vi "Teleop.vi"(10 "Match Info":T1={"Autonomous Elapsed Seconds"=0.0, "TeleOp Elapsed Seconds"=0.0, "Disabled Elapsed Seconds"=0.0, "Visited Autonomous"=FALSE, "Visited TeleOp"=FALSE, "Visited Disabled"=FALSE, "Autonomous Settings"={"Autonomous Style"=enum."Independent", "VI Refnum"=refnum}}, 11 "Call Context":T2) -> ()   [LabVIEW 2018]
doc: "This VI is called for each TeleOp packet received from the DS where the robot is not disabled. It is often used to read from the joysticks and update I/O or to update setpoints for timed control loops. It should complete and return within 20 milliseconds or it may miss DS packets."
uses:
  <vilib>/Rock Robotics/WPI/DriverStation/WPI_DriverStationDerivedRobotMode.ctl
  <vilib>/Rock Robotics/WPI/DriverStation/WPI_DriverStationMatch Info.ctl
  <vilib>/Rock Robotics/WPI/ThirdParty/Phoenix-LabVIEW/Motor Controller/Controls/CTRE_Phoenix_MotorControl_ControlMode.ctl
  <vilib>/Rock Robotics/WPI/Utilities/WPI_GetSetVariantRefNum.vi
  <vilib>/Rock Robotics/Network Tables/NT Write Boolean Array.vi
  <vilib>/Rock Robotics/Network Tables/NT Write Numeric Array.vi
  <vilib>/Rock Robotics/Network Tables/NT Write Number.vi
  Global 1.vi
panel:
  out "motor value after \nalex program":dbl
  out "slider value input":dbl
  # "r"
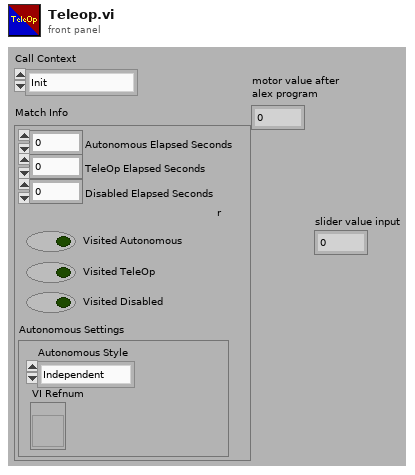
[diagram p1: front panel]
types:
  T1 = typedef "WPI_DriverStationMatch Info.ctl" = cluster{"Autonomous Elapsed Seconds":dbl, "TeleOp Elapsed Seconds":dbl, "Disabled Elapsed Seconds":dbl, "Visited Autonomous":bool, "Visited TeleOp":bool, "Visited Disabled":bool, "Autonomous Settings":cluster{"Autonomous Style":enum16{"Iterative", "Independent"}, "VI Refnum":refnum<vi>}}
  T2 = typedef "WPI_DriverStationDerivedRobotMode.ctl" = enum16{"Init", "Execute", "Stop"}
  T3 = typedef "WPI_JoystickDevRef.ctl" = cluster{"Device":T4}
  T4 = typedef "WPI_JoystickDeviceEnum.ctl" = enum16{"USB 0", "USB 1", "USB 2", "USB 3", "USB 4", "USB 5"}
  T5 = typedef "WPI_SwitchDevRef.ctl" = cluster{"DevStatus":errorcluster, "DIO Channel":T6, "CntIndex":T7, "Normally Closed":bool}
  T6 = typedef "FPGA_DIOChannel.ctl" = enum8{"DIO 0", "DIO 1", "DIO 2", "DIO 3", "DIO 4", "DIO 5", "DIO 6", "DIO 7", "DIO 8", "DIO 9", "DIO MXP 0", "DIO MXP 1", "DIO MXP 2", "DIO MXP 3", "DIO MXP 4", "DIO MXP 5", "DIO MXP 6", "DIO MXP 7", "DIO MXP 8", "DIO MXP 9", "DIO MXP 10", "DIO MXP 11", "DIO MXP 12", "DIO MXP 13", "DIO MXP 14", "DIO MXP 15", "SPI Port CS1", "SPI Port CS2", "SPI Port CS3", "SPI Port MISO", "SPI Port MOSI", "Invalid"}
  T7 = typedef "FPGA_CounterCtrSystemIndex.ctl" = enum8{"Ctr 0", "Ctr 1", "Ctr 2", "Ctr 3", "Ctr 4", "Ctr 5", "Ctr 6", "Ctr 7", "Invalid"}
  T8 = typedef "WPI_MotorControlDeviceRef.ctl" = cluster{"DeviceStatus":errorcluster, "Type":T9, "PWM":cluster{"PWM Channel":T10, "DeadBand":T11}, "CAN":cluster{"Device Number":u8, "SetOutput VI Ref":variant, "GetOutput VI Ref":variant, "Enable VI Ref":variant, "Disable VI Ref":variant, "Data":variant}, "Invert":bool, "DIO PWM":cluster{"PWM \"Enable\" Channel":T10, "DIOChannel":T6, "PWM Rate":dbl}}
  T9 = typedef "WPI_MotorControlType.ctl" = enum16{"PWM", "CAN", "DIO PWM"}
  T10 = typedef "FPGA_DIOPWMChannel.ctl" = enum8{"PWM 0", "PWM 1", "PWM 2", "PWM 3", "PWM 4", "PWM 5", "PWM 6", "PWM 7", "PWM 8", "PWM 9", "PWM MXP 0", "PWM MXP 1", "PWM MXP 2", "PWM MXP 3", "PWM MXP 4", "PWM MXP 5", "PWM MXP 6", "PWM MXP 7", "PWM MXP 8", "PWM MXP 9", "Invalid"}
  T11 = typedef "WPI_PWMDeadband.ctl" = cluster{"Name":string, "maxPositivePwm":i32, "minPositivePwm":i32, "centerPwm":i32, "maxNegativePwm":i32, "minNegativePwm":i32, "angularRange":u16}
  T12 = typedef "CTRE_Phoenix_MotorControl_ControlMode.ctl" = u16
  T13 = typedef "WPI_RobotDriveDevRef.ctl" = cluster{"DevStatus":errorcluster, "Motors[]":T8[], "Square Inputs":bool, "Max Output":dbl}
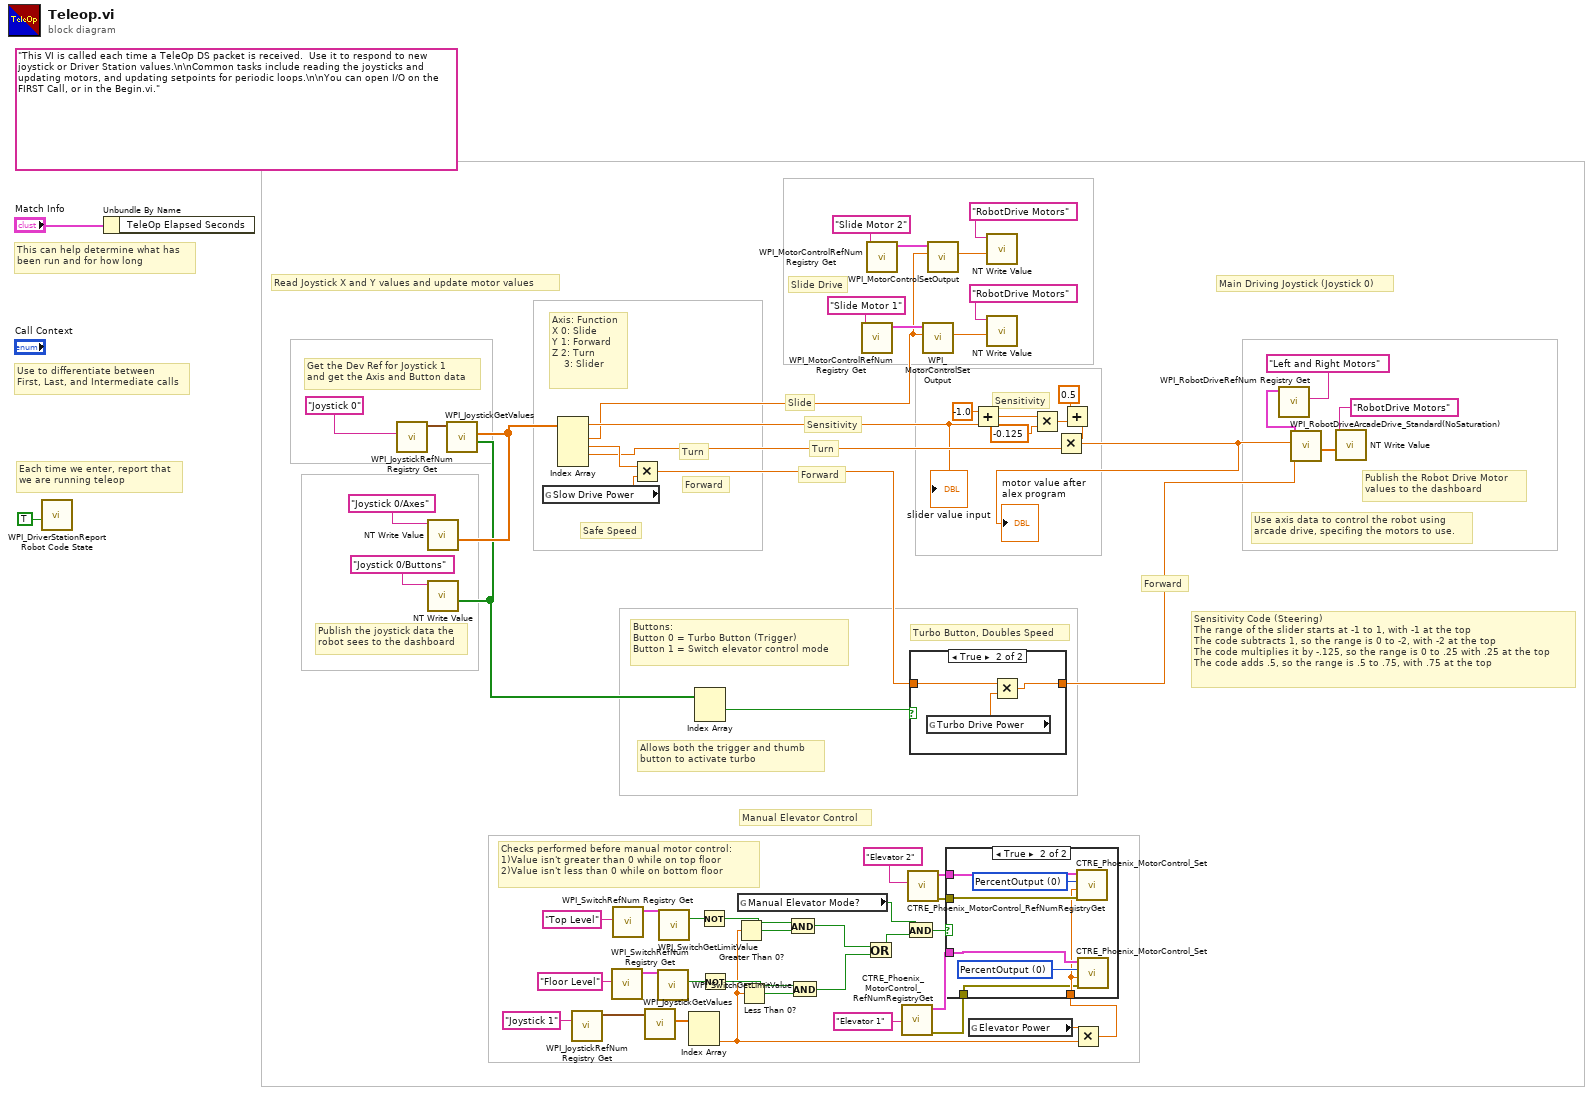
[diagram p0: block diagram]
diagram:
  (unwired) "This VI is called each time a TeleOp DS packet is received.  Use it to respond to new joystick or Driver Station values.\n\nCommon tasks include reading the joysticks and updating motors, and updating setpoints for periodic loops.\n\nYou can open I/O on the FIRST Call, or in the Begin.vi."
  # "Checks performed before manual motor control:\n1)Value isn't greater than 0 while on top floor\n2)Value isn't less than 0 while on bottom floor"
  # "Manual Elevator Control"
  # "Sensitivity Code (Steering)\nThe range of the slider starts at -1 to 1, with -1 at the top\nThe code subtracts 1, so the range is 0 to -2, with -2 at the top\nThe code multiplies it by -.125, so the range is 0 to .25 with .25 at the top\nThe code adds .5, so the range is .5 to .75, with .75 at the top"
  # "Sensitivity"
  # "Sensitivity"
  # "Allows both the trigger and thumb\nbutton to activate turbo"
  # "Slide Drive"
  # "Slide"
  # "Use axis data to control the robot using\narcade drive, specifing the motors to use."
  # "Get the Dev Ref for Joystick 1\nand get the Axis and Button data"
  # "Turn"
  # "Forward"
  # "Forward"
  # "Main Driving Joystick (Joystick 0)"
  # "Buttons:\nButton 0 = Turbo Button (Trigger)\nButton 1 = Switch elevator control mode"
  # "Safe Speed"
  # "Turbo Button, Doubles Speed"
  # "Forward"
  # "Turn"
  # "Axis: Function\nX 0: Slide \nY 1: Forward\nZ 2: Turn\n    3: Slider"
  # "Publish the Robot Drive Motor\nvalues to the dashboard"
  # "Publish the joystick data the\nrobot sees to the dashboard"
  # "Read Joystick X and Y values and update motor values"
  # "Each time we enter, report that\nwe are running teleop"
  # "Use to differentiate between\nFirst, Last, and Intermediate calls"
  # "This can help determine what has\nbeen run and for how long"
  n1 = call <vilib>:"WPI_DriverStationReport Robot Code State.vi"("TeleOp"=TRUE ("Autonomous")) -> ()  [unwired: 10 in, 1 out]
  n2 = Unbundle By Name("Match Info") -> ()  [unwired: 1 out]
  n3 = call <vilib>:"WPI_JoystickRefNum Registry Get.vi"("refnum name"="Joystick 0") -> ("JoystickDevRef"=w57:T3)  [unwired: 1 in, 9 out]
  n4 = call <vilib>:"WPI_JoystickGetValues.vi"("JoystickDevRef"=w57) -> ("Buttons"=w48:bool[], "Axes"=w54:dbl[])  [unwired: 6 in, 3 out]
  n5 = call-poly <vilib>:"NT Write Value.vi"("Numeric Array"=w54, "Name"="Joystick 0/Axes") -> ()  [unwired: 9 in, 1 out]
  n6 = call-poly <vilib>:"NT Write Value.vi"("Boolean Array"=w48, "Name"="Joystick 0/Buttons") -> ()  [unwired: 9 in, 1 out]
  n7 = global read "Global 1.vi" "Slow Drive Power"() -> (w37:dbl)
  n8 = Index Array(array=w54) -> (element #1=w4:dbl, element #2=w49:dbl, element #3=w40:dbl, element #4=w39:dbl)  [unwired: 4 in]
  "slider value input" <- w39
  n9 = call <vilib>:"WPI_JoystickRefNum Registry Get.vi"("refnum name"="Joystick 1") -> ("JoystickDevRef"=w23:T3)  [unwired: 1 in, 9 out]
  n10 = call <vilib>:"WPI_SwitchRefNum Registry Get.vi"("refnum name"="Floor Level") -> ("SwitchDevRef"=w33:T5)  [unwired: 9 in, 1 out]
  n11 = call <vilib>:"WPI_SwitchRefNum Registry Get.vi"("refnum name"="Top Level") -> ("SwitchDevRef"=w32:T5)  [unwired: 9 in, 1 out]
  n12 = Multiply(x=w49, y=w37) -> (x*y=w51:dbl)
  n13 = call <vilib>:"WPI_JoystickGetValues.vi"("JoystickDevRef"=w23) -> ("Axes"=w29:dbl[])  [unwired: 6 in, 4 out]
  n14 = call <vilib>:"WPI_SwitchGetLimitValue.vi"("SwitchDevRef"=w33) -> ("Switch Pressed"=w31:bool)  [unwired: 8 in, 2 out]
  n15 = call <vilib>:"WPI_SwitchGetLimitValue.vi"("SwitchDevRef"=w32) -> ("Switch Pressed"=w30:bool)  [unwired: 8 in, 2 out]
  n16 = Index Array(array=w29) -> (element #2=w10:dbl)  [unwired: 2 in, 1 out]
  n17 = Index Array(array=w48) -> (element #1=w36:bool)  [unwired: 2 in, 1 out]
  n18 = Not(x=w30) -> (.not. x?=w19:bool)
  n19 = Not(x=w31) -> (.not. x?=w18:bool)
  n20 = Greater Than 0?(x=w10) -> (x > 0?=w21:bool)
  n21 = global read "Global 1.vi" "Manual Elevator Mode?"() -> (w22:bool)
  n22 = Less Than 0?(x=w10) -> (x < 0?=w20:bool)
  n23 = And(x=w19, y=w21) -> (x .and. y?=w14:bool)
  n24 = And(x=w18, y=w20) -> (x .and. y?=w11:bool)
  n25 = call <vilib>:"WPI_MotorControlRefNum Registry Get.vi"("refnum name"="Slide Motor 1") -> ("MotorControlDevRef"=w46:T8)  [unwired: 9 in, 1 out]
  n26 = Or(x=w14, y=w11) -> (x .or. y?=w12:bool)
  n27 = call <vilib>:"WPI_MotorControlRefNum Registry Get.vi"("refnum name"="Slide Motor 2") -> ("MotorControlDevRef"=w5:T8)  [unwired: 9 in, 1 out]
  n28 = call <vilib>:"CTRE_Phoenix_MotorControl_RefNumRegistryGet.vi"("refnum name"="Elevator 1") -> ("error out"=w1:errorcluster, "PhoenixMotorControlDevRef"=w27:T8)  [unwired: 9 in]
  n29 = And(x=w22, y=w12) -> (x .and. y?=w13:bool)
  n30 = call <vilib>:"CTRE_Phoenix_MotorControl_RefNumRegistryGet.vi"("refnum name"="Elevator 2") -> ("error out"=w7:errorcluster, "PhoenixMotorControlDevRef"=w8:T8)  [unwired: 9 in]
  n31 = case shown="True" w36 {
    tunnel: w51 -> [w63 w66]
    tunnel: [w63 w65] -> w50
    frame False {
    }
    frame True {
      n32 = global read "Global 1.vi" "Turbo Drive Power"() -> (w64:dbl)
      n33 = Multiply(x=w66, y=w64) -> (x*y=w65:dbl)
    }
  }
  n34 = call <vilib>:"WPI_MotorControlSetOutput.vi"("Output"=w4, "MotorControlDevRef"=w46) -> ("Motor Output"=w45:dbl)  [unwired: 7 in, 2 out]
  n35 = call <vilib>:"WPI_MotorControlSetOutput.vi"("Output"=w4, "MotorControlDevRef"=w5) -> ("Motor Output"=w2:dbl)  [unwired: 7 in, 2 out]
  n36 = global read "Global 1.vi" "Elevator Power"() -> (w25:dbl)
  n37 = Add(x=-1.0, y=w39) -> (x+y=w42:dbl)
  n38 = call-poly <vilib>:"NT Write Value.vi"("Numeric"=w2, "Name"="RobotDrive Motors" ("refnum name")) -> ()  [unwired: 9 in, 1 out]
  n39 = call-poly <vilib>:"NT Write Value.vi"("Numeric"=w45, "Name"="RobotDrive Motors" ("refnum name")) -> ()  [unwired: 9 in, 1 out]
  n40 = Multiply(x=w42, y=-0.125) -> (x*y=w16:dbl)
  n41 = Add(x=0.5, y=w16) -> (x+y=w17:dbl)
  n42 = Multiply(x=w17, y=w40) -> (x*y=w38:dbl)
  "motor value after \nalex program" <- w38
  n43 = Multiply(x=w25, y=w10) -> (x*y=w26:dbl)
  n44 = case shown="True" w13 {
    tunnel: w26 -> [_ w69]
    tunnel: w27 -> [_ w72]
    tunnel: w8 -> [_ w71]
    tunnel: w7 -> [_ w70]
    tunnel: w1 -> [_ w67]
    frame False {
    }
    frame True {
      w68 = T12 0 items=["PercentOutput"=0, "Position"=1, "Velocity"=2, "Current"=3, "Follower"=5, "MotionProfile"=6, "MotionMagic"=7, "MotionProfileArc"=10, "Disabled"=15] ("Control Mode")
      w73 = T12 0 items=["PercentOutput"=0, "Position"=1, "Velocity"=2, "Current"=3, "Follower"=5, "MotionProfile"=6, "MotionMagic"=7, "MotionProfileArc"=10, "Disabled"=15] ("Control Mode")
      n45 = call <vilib>:"CTRE_Phoenix_MotorControl_Set.vi"("error in (no error)"=w70, "Output"=w69, "Control Mode"=w68, "PhoenixMotorControlDevRef"=w71) -> ()  [unwired: 6 in, 2 out]
      n46 = call <vilib>:"CTRE_Phoenix_MotorControl_Set.vi"("error in (no error)"=w67, "Output"=w69, "Control Mode"=w73, "PhoenixMotorControlDevRef"=w72) -> ()  [unwired: 6 in, 2 out]
    }
  }
  n47 = call <vilib>:"WPI_RobotDriveRefNum Registry Get.vi"("refnum name"="Left and Right Motors") -> ("RobotDriveDevRef"=w59:T13)  [unwired: 1 in, 9 out]
  n48 = call <vilib>:"WPI_RobotDriveArcadeDrive_Standard(NoSaturation).vi"("Y axis value"=w50, "X axis value"=w38, "RobotDriveDevRef"=w59) -> ("Motor Values"=w53:dbl[])  [unwired: 1 in, 7 out]
  n49 = call-poly <vilib>:"NT Write Value.vi"("Numeric Array"=w53, "Name"="RobotDrive Motors") -> ()  [unwired: 9 in, 1 out]
